vi "Test_Check_Group_Edges_Caraya.vi"(8 "error in":errorcluster) -> (0 "error out":errorcluster)   [LabVIEW 2026]
doc: "Caraya edge cases for the configurable step checks: AND/OR combinations, inclusive range limits, compare modes and first-failure reporting."
uses:
  <vilib>/addons/_JKI Toolkits/Caraya/classes/Test/Test.lvclass
  <vilib>/addons/_JKI Toolkits/Caraya/classes/Assert/Assert.lvclass
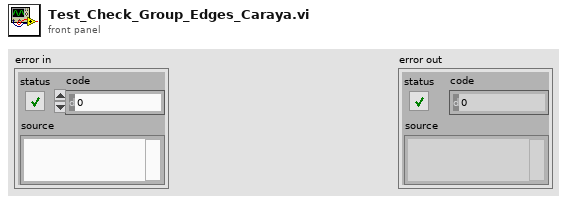
[diagram p1: front panel]
types:
  T1 = cluster{"di_high":cluster{"and_list":string[], "or_list":string[]}, "di_low":cluster{"and_list":string[], "or_list":string[]}, "misc_high":cluster{"and_list":string[], "or_list":string[]}, "misc_low":cluster{"and_list":string[], "or_list":string[]}, "t0_high":cluster{"and_list":cluster{"name":string, "min":dbl, "max":dbl}[], "or_list":cluster{"name":string, "min":dbl, "max":dbl}[]}, "t0_low":cluster{"and_list":cluster{"name":string, "min":dbl, "max":dbl}[], "or_list":cluster{"name":string, "min":dbl, "max":dbl}[]}, "misc_compare":cluster{"name":string, "compare_with":string, "comparison":enum16{"EQ", "NE", "GT", "GE", "LT", "LE"}, "tolerance":dbl}[]}
  T2 = cluster{"name":string, "compare_with":string, "comparison":enum16{"EQ", "NE", "GT", "GE", "LT", "LE"}, "tolerance":dbl}[]
  T3 = cluster{"and_list":cluster{"name":string, "min":dbl, "max":dbl}[], "or_list":cluster{"name":string, "min":dbl, "max":dbl}[]}
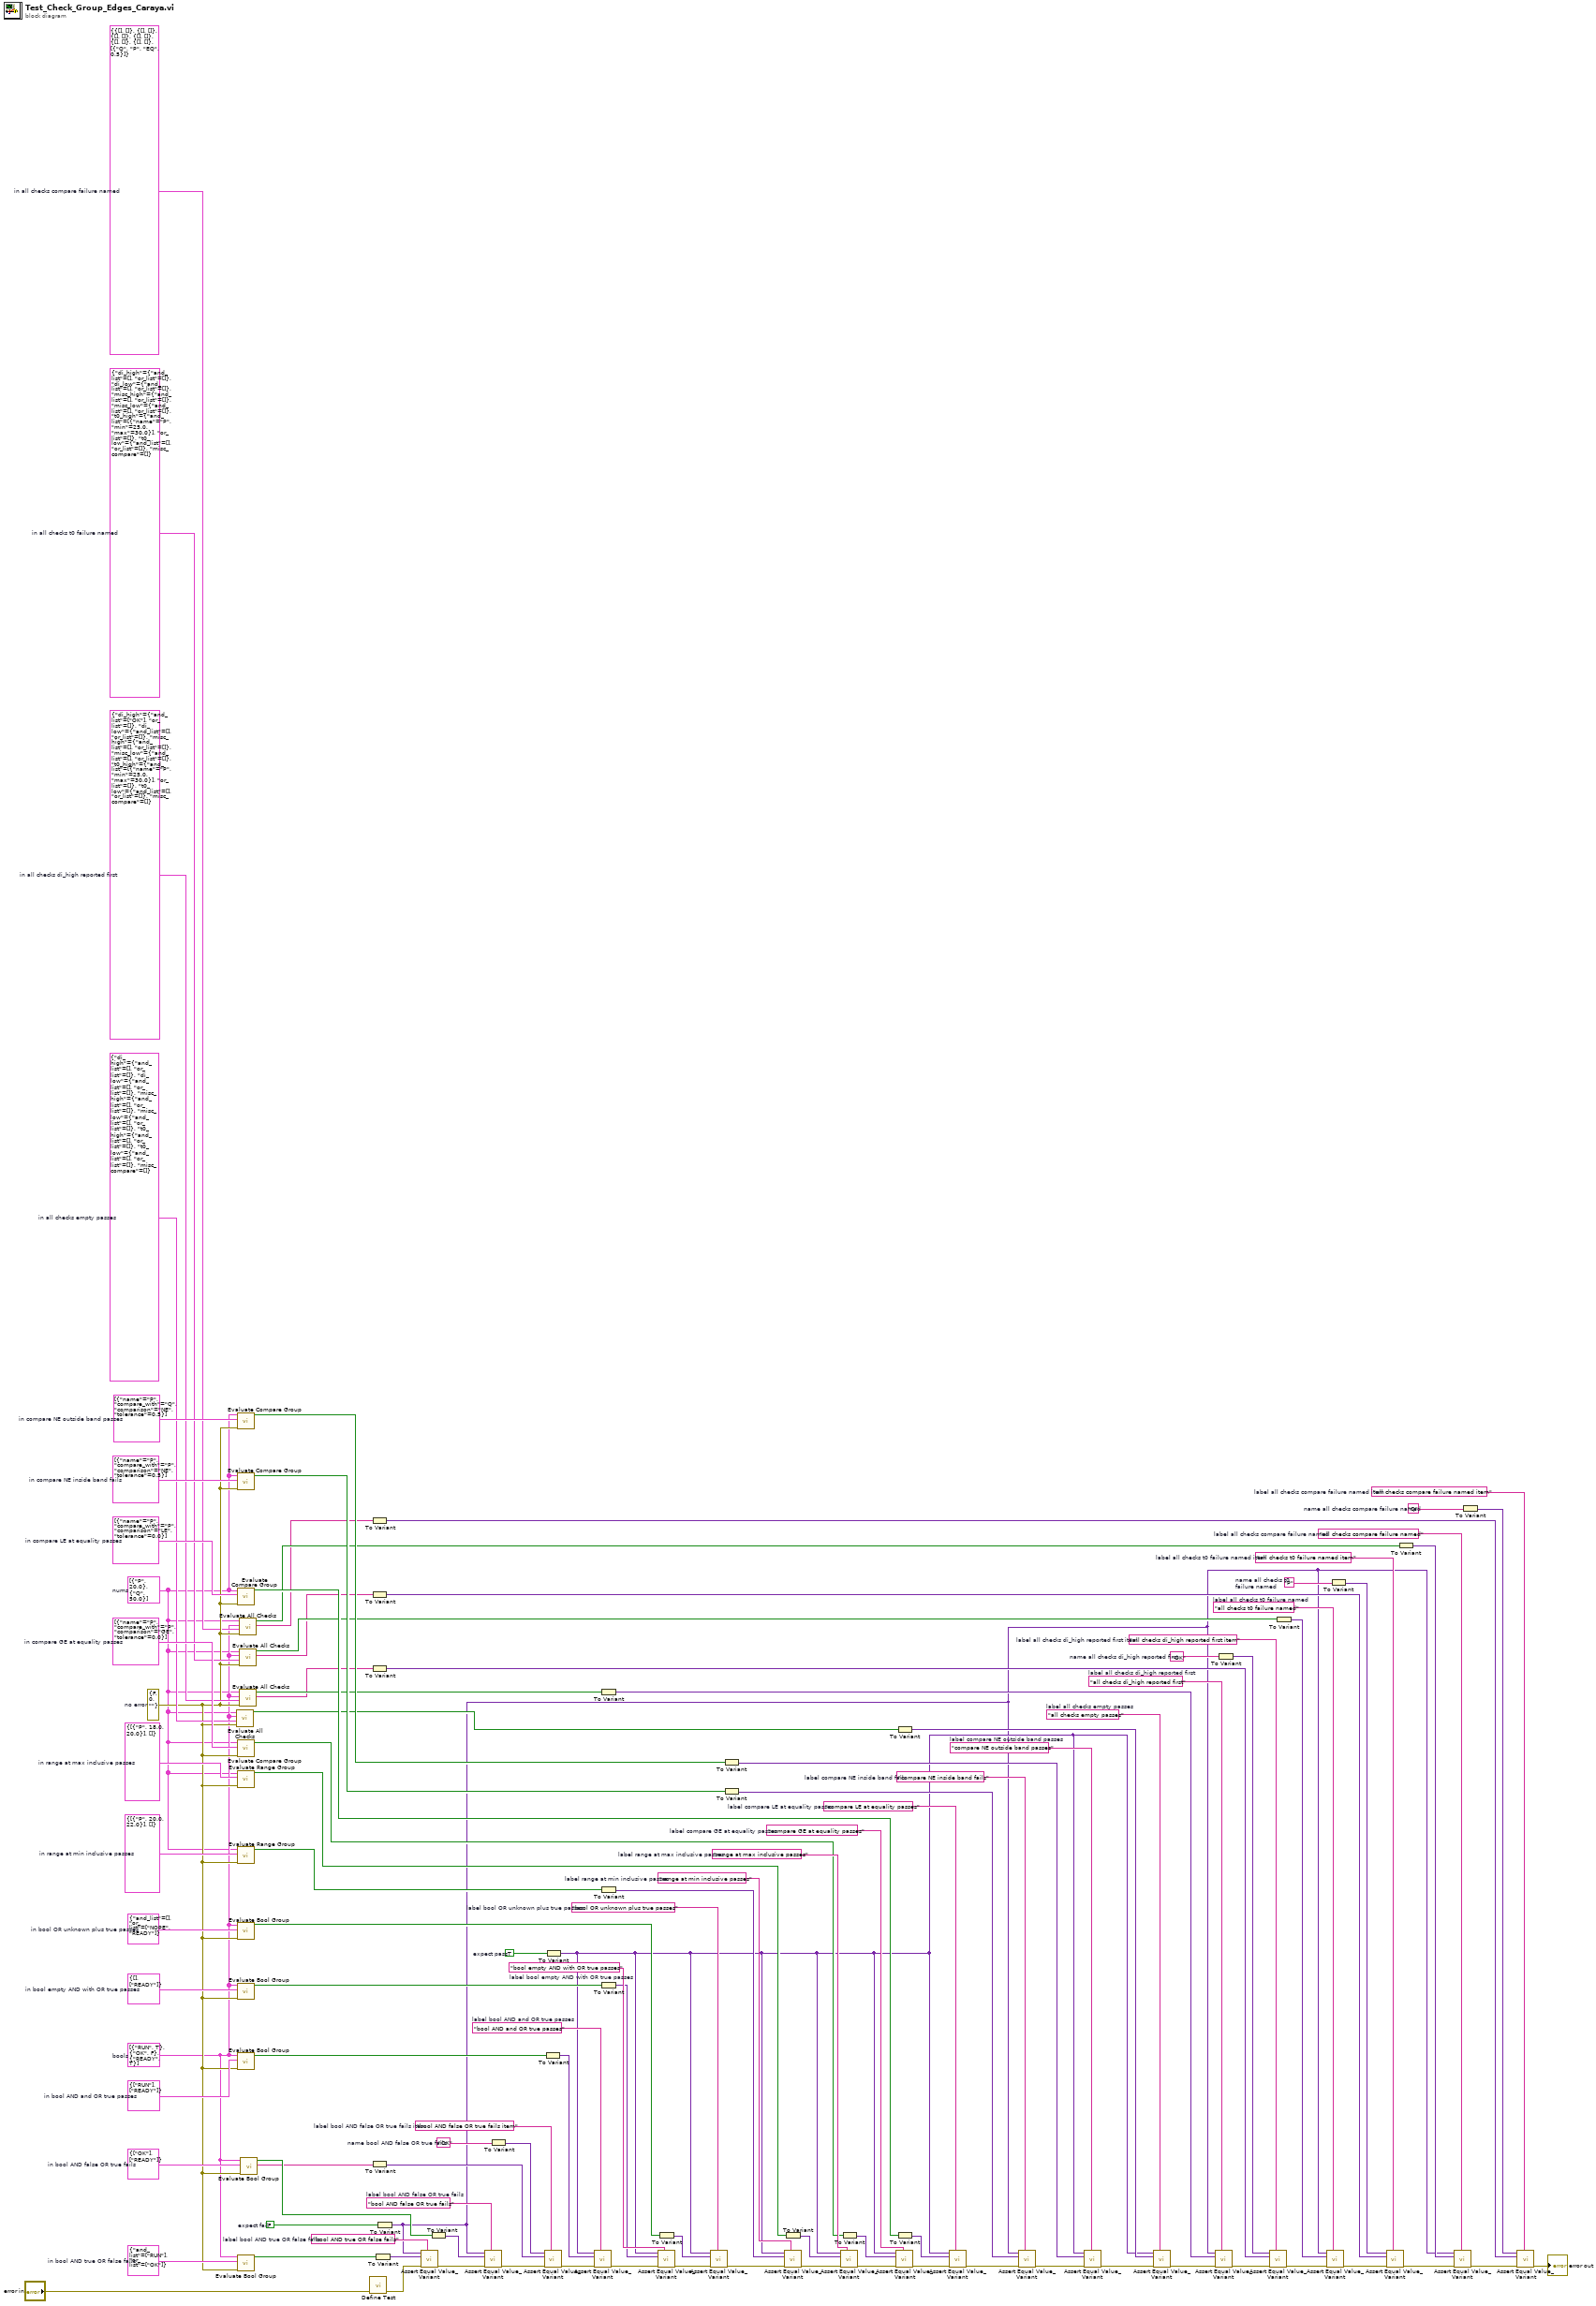
[diagram p0: block diagram]
diagram:
  w5 = "all checks compare failure named item"  # label all checks compare failure named item
  w6 = "Q"  # name all checks compare failure named
  w11 = "all checks compare failure named"  # label all checks compare failure named
  w15 = T1 {"di_high"={"and_list"=[], "or_list"=[]}, "di_low"={"and_list"=[], "or_list"=[]}, "misc_high"={"and_list"=[], "or_list"=[]}, "misc_low"={"and_list"=[], "or_list"=[]}, "t0_high"={"and_list"=[], "or_list"=[]}, "t0_low"={"and_list"=[], "or_list"=[]}, "misc_compare"=[{"name"="Q", "compare_with"="P", "comparison"=enum."EQ", "tolerance"=0.5}]}  # in all checks compare failure named
  w20 = "all checks t0 failure named item"  # label all checks t0 failure named item
  w21 = "P"  # name all checks t0 failure named
  w25 = "all checks t0 failure named"  # label all checks t0 failure named
  w27 = T1 {"di_high"={"and_list"=[], "or_list"=[]}, "di_low"={"and_list"=[], "or_list"=[]}, "misc_high"={"and_list"=[], "or_list"=[]}, "misc_low"={"and_list"=[], "or_list"=[]}, "t0_high"={"and_list"=[{"name"="P", "min"=25.0, "max"=30.0}], "or_list"=[]}, "t0_low"={"and_list"=[], "or_list"=[]}, "misc_compare"=[]}  # in all checks t0 failure named
  w31 = "all checks di_high reported first item"  # label all checks di_high reported first item
  w32 = "OK"  # name all checks di_high reported first
  w36 = "all checks di_high reported first"  # label all checks di_high reported first
  w38 = T1 {"di_high"={"and_list"=["OK"], "or_list"=[]}, "di_low"={"and_list"=[], "or_list"=[]}, "misc_high"={"and_list"=[], "or_list"=[]}, "misc_low"={"and_list"=[], "or_list"=[]}, "t0_high"={"and_list"=[{"name"="P", "min"=25.0, "max"=30.0}], "or_list"=[]}, "t0_low"={"and_list"=[], "or_list"=[]}, "misc_compare"=[]}  # in all checks di_high reported first
  w42 = "all checks empty passes"  # label all checks empty passes
  w44 = T1 {"di_high"={"and_list"=[], "or_list"=[]}, "di_low"={"and_list"=[], "or_list"=[]}, "misc_high"={"and_list"=[], "or_list"=[]}, "misc_low"={"and_list"=[], "or_list"=[]}, "t0_high"={"and_list"=[], "or_list"=[]}, "t0_low"={"and_list"=[], "or_list"=[]}, "misc_compare"=[]}  # in all checks empty passes
  w47 = "compare NE outside band passes"  # label compare NE outside band passes
  w49 = T2 [{"name"="P", "compare_with"="Q", "comparison"=enum."NE", "tolerance"=0.5}]  # in compare NE outside band passes
  w52 = "compare NE inside band fails"  # label compare NE inside band fails
  w54 = T2 [{"name"="P", "compare_with"="P", "comparison"=enum."NE", "tolerance"=0.5}]  # in compare NE inside band fails
  w57 = "compare LE at equality passes"  # label compare LE at equality passes
  w59 = T2 [{"name"="P", "compare_with"="P", "comparison"=enum."LE", "tolerance"=0.0}]  # in compare LE at equality passes
  w62 = "compare GE at equality passes"  # label compare GE at equality passes
  w64 = T2 [{"name"="P", "compare_with"="P", "comparison"=enum."GE", "tolerance"=0.0}]  # in compare GE at equality passes
  w67 = "range at max inclusive passes"  # label range at max inclusive passes
  w69 = T3 {"and_list"=[{"name"="P", "min"=18.0, "max"=20.0}], "or_list"=[]}  # in range at max inclusive passes
  w72 = "range at min inclusive passes"  # label range at min inclusive passes
  w74 = T3 {"and_list"=[{"name"="P", "min"=20.0, "max"=22.0}], "or_list"=[]}  # in range at min inclusive passes
  w77 = "bool OR unknown plus true passes"  # label bool OR unknown plus true passes
  w79 = cluster{"and_list":string[], "or_list":string[]} {"and_list"=[], "or_list"=["NOPE", "READY"]}  # in bool OR unknown plus true passes
  w82 = "bool empty AND with OR true passes"  # label bool empty AND with OR true passes
  w84 = cluster{"and_list":string[], "or_list":string[]} {"and_list"=[], "or_list"=["READY"]}  # in bool empty AND with OR true passes
  w87 = "bool AND and OR true passes"  # label bool AND and OR true passes
  w89 = cluster{"and_list":string[], "or_list":string[]} {"and_list"=["RUN"], "or_list"=["READY"]}  # in bool AND and OR true passes
  w93 = "bool AND false OR true fails item"  # label bool AND false OR true fails item
  w94 = "OK"  # name bool AND false OR true fails
  w98 = "bool AND false OR true fails"  # label bool AND false OR true fails
  w100 = cluster{"and_list":string[], "or_list":string[]} {"and_list"=["OK"], "or_list"=["READY"]}  # in bool AND false OR true fails
  w103 = "bool AND true OR false fails"  # label bool AND true OR false fails
  w105 = cluster{"and_list":string[], "or_list":string[]} {"and_list"=["RUN"], "or_list"=["OK"]}  # in bool AND true OR false fails
  w107 = FALSE  # expect fail
  w108 = TRUE  # expect pass
  w13 = cluster{"channel":string, "value":dbl}[] [{"channel"="P", "value"=20.0}, {"channel"="Q", "value"=50.0}]  # nums
  w14 = cluster{"name":string, "on":bool}[] [{"name"="RUN", "on"=TRUE}, {"name"="OK", "on"=FALSE}, {"name"="READY", "on"=TRUE}]  # bools
  w16 = errorcluster {"status"=FALSE, "code"=0, "source"=""}  # no error
  n1 = call "Evaluate All Checks.vi"("error in"=w16, "checks"=w44, "bool values"=w14, "num values"=w13) -> ("passes"=w43:bool)  [unwired: 5 in, 2 out]
  n2 = call "Evaluate Compare Group.vi"("error in"=w16, "items"=w49, "num values"=w13) -> ("passes"=w48:bool)  [unwired: 6 in, 2 out]
  n3 = call "Evaluate Compare Group.vi"("error in"=w16, "items"=w54, "num values"=w13) -> ("passes"=w53:bool)  [unwired: 6 in, 2 out]
  n4 = call "Evaluate Compare Group.vi"("error in"=w16, "items"=w59, "num values"=w13) -> ("passes"=w58:bool)  [unwired: 6 in, 2 out]
  n5 = call "Evaluate Compare Group.vi"("error in"=w16, "items"=w64, "num values"=w13) -> ("passes"=w63:bool)  [unwired: 6 in, 2 out]
  n6 = call "Evaluate Range Group.vi"("error in"=w16, "group"=w69, "num values"=w13) -> ("passes"=w68:bool)  [unwired: 6 in, 2 out]
  n7 = call "Evaluate Range Group.vi"("error in"=w16, "group"=w74, "num values"=w13) -> ("passes"=w73:bool)  [unwired: 6 in, 2 out]
  n8 = call "Evaluate Bool Group.vi"("error in"=w16, "group"=w79, "bool values"=w14) -> ("passes"=w78:bool)  [unwired: 6 in, 2 out]
  n9 = call "Evaluate Bool Group.vi"("error in"=w16, "group"=w84, "bool values"=w14) -> ("passes"=w83:bool)  [unwired: 6 in, 2 out]
  n10 = call "Evaluate Bool Group.vi"("error in"=w16, "group"=w89, "bool values"=w14) -> ("passes"=w88:bool)  [unwired: 6 in, 2 out]
  n11 = call "Evaluate Bool Group.vi"("error in"=w16, "group"=w105, "bool values"=w14) -> ("passes"=w104:bool)  [unwired: 6 in, 2 out]
  n12 = call "Evaluate All Checks.vi"("error in"=w16, "checks"=w15, "bool values"=w14, "num values"=w13) -> ("first fail"=w7:string, "passes"=w12:bool)  [unwired: 5 in, 1 out]
  n13 = call "Evaluate All Checks.vi"("error in"=w16, "checks"=w27, "bool values"=w14, "num values"=w13) -> ("first fail"=w22:string, "passes"=w26:bool)  [unwired: 5 in, 1 out]
  n14 = call "Evaluate All Checks.vi"("error in"=w16, "checks"=w38, "bool values"=w14, "num values"=w13) -> ("first fail"=w33:string, "passes"=w37:bool)  [unwired: 5 in, 1 out]
  n15 = call "Evaluate Bool Group.vi"("error in"=w16, "group"=w100, "bool values"=w14) -> ("first fail"=w95:string, "passes"=w99:bool)  [unwired: 6 in, 1 out]
  n16 = call <vilib>:"Define Test.vi"("error in (no error)"="error in") -> ("error out"=w102:errorcluster)  [unwired: 9 in, 1 out]
  n17 = To Variant(anything=w7) -> (Variant=w3:variant)
  n18 = To Variant(anything=w22) -> (Variant=w18:variant)
  n19 = To Variant(anything=w33) -> (Variant=w29:variant)
  n20 = To Variant(anything=w95) -> (Variant=w91:variant)
  n21 = To Variant(anything=w104) -> (Variant=w101:variant)
  n22 = To Variant(anything=w107) -> (Variant=w8:variant)
  n23 = call <vilib>:"Assert Equal Value_Variant.vi"("Label"=w103, "error in (no error)"=w102, "Actual"=w101, "Expected"=w8) -> ("error out"=w97:errorcluster)  [unwired: 6 in, 1 out]
  n24 = To Variant(anything=w99) -> (Variant=w96:variant)
  n25 = call <vilib>:"Assert Equal Value_Variant.vi"("Label"=w98, "error in (no error)"=w97, "Actual"=w96, "Expected"=w8) -> ("error out"=w92:errorcluster)  [unwired: 6 in, 1 out]
  n26 = To Variant(anything=w94) -> (Variant=w90:variant)
  n27 = call <vilib>:"Assert Equal Value_Variant.vi"("Label"=w93, "error in (no error)"=w92, "Actual"=w91, "Expected"=w90) -> ("error out"=w86:errorcluster)  [unwired: 6 in, 1 out]
  n28 = To Variant(anything=w88) -> (Variant=w85:variant)
  n29 = To Variant(anything=w108) -> (Variant=w39:variant)
  n30 = call <vilib>:"Assert Equal Value_Variant.vi"("Label"=w87, "error in (no error)"=w86, "Actual"=w85, "Expected"=w39) -> ("error out"=w81:errorcluster)  [unwired: 6 in, 1 out]
  n31 = To Variant(anything=w37) -> (Variant=w34:variant)
  n32 = To Variant(anything=w73) -> (Variant=w70:variant)
  n33 = To Variant(anything=w83) -> (Variant=w80:variant)
  n34 = call <vilib>:"Assert Equal Value_Variant.vi"("Label"=w82, "error in (no error)"=w81, "Actual"=w80, "Expected"=w39) -> ("error out"=w76:errorcluster)  [unwired: 6 in, 1 out]
  n35 = To Variant(anything=w78) -> (Variant=w75:variant)
  n36 = call <vilib>:"Assert Equal Value_Variant.vi"("Label"=w77, "error in (no error)"=w76, "Actual"=w75, "Expected"=w39) -> ("error out"=w71:errorcluster)  [unwired: 6 in, 1 out]
  n37 = To Variant(anything=w48) -> (Variant=w45:variant)
  n38 = To Variant(anything=w53) -> (Variant=w50:variant)
  n39 = call <vilib>:"Assert Equal Value_Variant.vi"("Label"=w72, "error in (no error)"=w71, "Actual"=w70, "Expected"=w39) -> ("error out"=w66:errorcluster)  [unwired: 6 in, 1 out]
  n40 = To Variant(anything=w68) -> (Variant=w65:variant)
  n41 = call <vilib>:"Assert Equal Value_Variant.vi"("Label"=w67, "error in (no error)"=w66, "Actual"=w65, "Expected"=w39) -> ("error out"=w61:errorcluster)  [unwired: 6 in, 1 out]
  n42 = To Variant(anything=w63) -> (Variant=w60:variant)
  n43 = call <vilib>:"Assert Equal Value_Variant.vi"("Label"=w62, "error in (no error)"=w61, "Actual"=w60, "Expected"=w39) -> ("error out"=w56:errorcluster)  [unwired: 6 in, 1 out]
  n44 = To Variant(anything=w43) -> (Variant=w40:variant)
  n45 = To Variant(anything=w58) -> (Variant=w55:variant)
  n46 = call <vilib>:"Assert Equal Value_Variant.vi"("Label"=w57, "error in (no error)"=w56, "Actual"=w55, "Expected"=w39) -> ("error out"=w51:errorcluster)  [unwired: 6 in, 1 out]
  n47 = call <vilib>:"Assert Equal Value_Variant.vi"("Label"=w52, "error in (no error)"=w51, "Actual"=w50, "Expected"=w8) -> ("error out"=w46:errorcluster)  [unwired: 6 in, 1 out]
  n48 = call <vilib>:"Assert Equal Value_Variant.vi"("Label"=w47, "error in (no error)"=w46, "Actual"=w45, "Expected"=w39) -> ("error out"=w41:errorcluster)  [unwired: 6 in, 1 out]
  n49 = call <vilib>:"Assert Equal Value_Variant.vi"("Label"=w42, "error in (no error)"=w41, "Actual"=w40, "Expected"=w39) -> ("error out"=w35:errorcluster)  [unwired: 6 in, 1 out]
  n50 = call <vilib>:"Assert Equal Value_Variant.vi"("Label"=w36, "error in (no error)"=w35, "Actual"=w34, "Expected"=w8) -> ("error out"=w30:errorcluster)  [unwired: 6 in, 1 out]
  n51 = To Variant(anything=w32) -> (Variant=w28:variant)
  n52 = call <vilib>:"Assert Equal Value_Variant.vi"("Label"=w31, "error in (no error)"=w30, "Actual"=w29, "Expected"=w28) -> ("error out"=w24:errorcluster)  [unwired: 6 in, 1 out]
  n53 = To Variant(anything=w26) -> (Variant=w23:variant)
  n54 = call <vilib>:"Assert Equal Value_Variant.vi"("Label"=w25, "error in (no error)"=w24, "Actual"=w23, "Expected"=w8) -> ("error out"=w19:errorcluster)  [unwired: 6 in, 1 out]
  n55 = To Variant(anything=w21) -> (Variant=w17:variant)
  n56 = call <vilib>:"Assert Equal Value_Variant.vi"("Label"=w20, "error in (no error)"=w19, "Actual"=w18, "Expected"=w17) -> ("error out"=w10:errorcluster)  [unwired: 6 in, 1 out]
  n57 = To Variant(anything=w12) -> (Variant=w9:variant)
  n58 = call <vilib>:"Assert Equal Value_Variant.vi"("Label"=w11, "error in (no error)"=w10, "Actual"=w9, "Expected"=w8) -> ("error out"=w4:errorcluster)  [unwired: 6 in, 1 out]
  n59 = To Variant(anything=w6) -> (Variant=w2:variant)
  n60 = call <vilib>:"Assert Equal Value_Variant.vi"("Label"=w5, "error in (no error)"=w4, "Actual"=w3, "Expected"=w2) -> ("error out"=→"error out":errorcluster)  [unwired: 6 in, 1 out]
